vi "Set Output.vi"(8 "error in (no error)":errorcluster, 9 "Set Output":bool, 10 "DIO_CFG":refnum<class "DIO-Configuration.lvclass">, 11 "UI Template in":refnum<class "DIO_Panel.lvclass">) -> (0 "error out":errorcluster, 3 "UI Template out":refnum<class "DIO_Panel.lvclass">)   [LabVIEW 2021, in "Simulator-Channel.lvlib" / "DIO_Panel.lvlib" / "DIO_Panel.lvclass"]
uses:
  DIO_Panel.lvclass
  Dependencies/DIO-Channel.lvlibp/Channels/DIO-Channel/DIO-Configuration_class/DIO-Configuration.lvclass
  C:/Users/averna/Documents/LV Gym DEMO/Factory Pattern/Channels/Dependencies/Channel.lvlibp/Channel/Configuration_class/Configuration.lvclass
  DIO_Panel.lvclass/DIO_Panel.ctl
  tdef/info.ctl
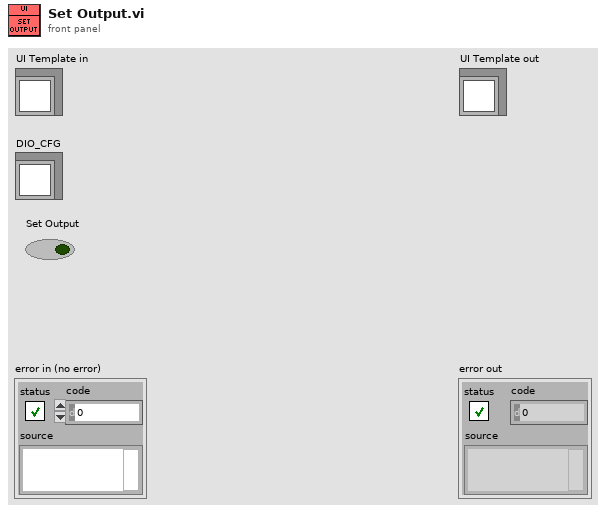
[diagram p1: front panel]
types:
  T1 = typedef "Simulator-Channel.lvlib/DIO_Panel.lvlib/DIO_Panel.lvclass/info.ctl" = cluster{"Name":string, "Boolean":bool}
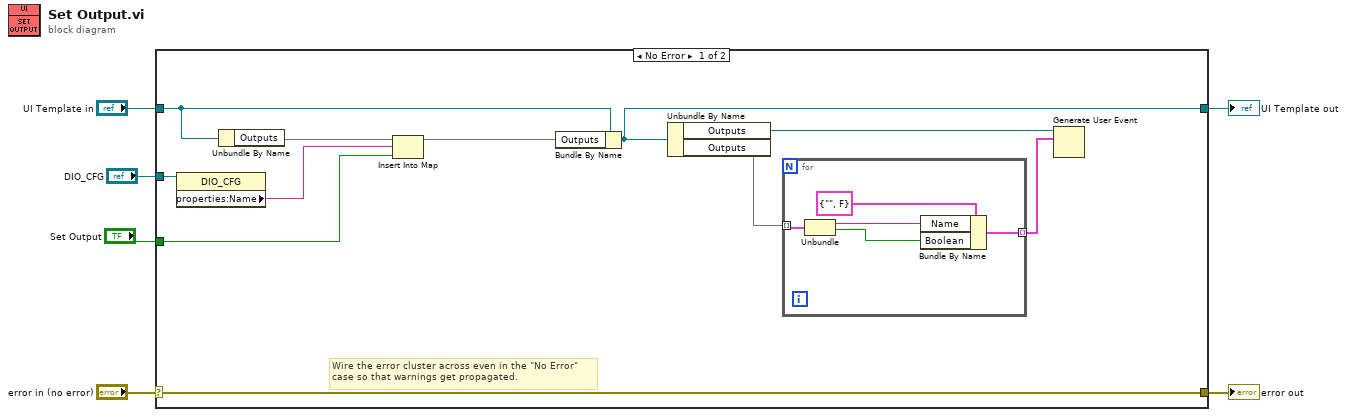
[diagram p0: block diagram]
diagram:
  n1 = case shown="No Error" "error in (no error)" {
    selector: "error in (no error)" -> [w17 w24]
    tunnel: [w17 w24] -> w5
    tunnel: [w10 w23] -> w3
    tunnel: "UI Template in" -> [w16 w23]
    tunnel: "Set Output" -> [w13 _]
    tunnel: "DIO_CFG" -> [w12 _]
    frame No Error {
      # "Wire the error cluster across even in the \"No Error\"\ncase so that warnings get propagated."
      n2 = property class="DIO_CFG"(reference=w12) -> ("properties:Name"=w11:string)  [unwired: 1 in, 2 out]
      n3 = Unbundle By Name(w16) -> ("Outputs"=w15:map{string, bool})
      n4 = Insert Into Map(map in=w15, key=w11, value=w13) -> (map out=w14:map{string, bool})  [unwired: 2 out]
      n5 = Bundle By Name(cluster=w16, "Outputs"=w14) -> (w10:refnum<class "DIO_Panel.lvclass">)
      n6 = Unbundle By Name(w10) -> ("Outputs"=w8:refnum<user-event>, "Outputs"=w9:map{string, bool})
      n7 = for {
        tunnel: w9 -> [w22] mode=indexing
        tunnel: [w18] -> w7 mode=indexing
        n8 = Unbundle(w22) -> (w20:string, "Boolean"=w19:bool)
        n9 = Bundle By Name(cluster=T1 {"Name"="", "Boolean"=FALSE} ("Info"), "Name"=w20, "Boolean"=w19) -> (w18:T1)
      }
      n10 = Generate User Event(user event=w8, event data cluster=w7) -> ()  [unwired: 2 in, 2 out]
    }
    frame Error {
    }
  }
  "error out" <- w5
  "UI Template out" <- w3
